vi "Units_to_Pa.vi"(1 "Units":enum16{"psi", "bar", "kPa", "Pa"}(ring)=enum."Pa", 2 "Value":dbl) -> (0 "P_Pa":dbl)   [LabVIEW 2025]
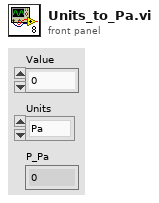
[diagram p1: front panel]
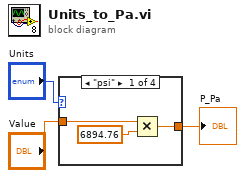
[diagram p0: block diagram]
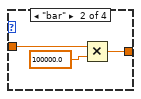
[diagram p2: hidden frame]
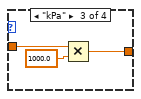
[diagram p3: hidden frame]
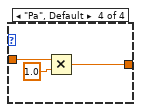
[diagram p4: hidden frame]
diagram:
  n1 = case shown="\"psi\"" "Units" {
    tunnel: "Value" -> [w4 w7 w11 w14]
    tunnel: [w5 w8 w10 w13] -> w1
    frame "psi" {
      n2 = Multiply(x=w4, y=6894.76) -> (x*y=w5:dbl)
    }
    frame "bar" {
      n3 = Multiply(x=w7, y=100000.0) -> (x*y=w8:dbl)
    }
    frame "kPa" {
      n4 = Multiply(x=w11, y=1000.0) -> (x*y=w10:dbl)
    }
    frame "Pa", Default {
      n5 = Multiply(x=w14, y=1.0) -> (x*y=w13:dbl)
    }
  }
  "P_Pa" <- w1
